vi "CalcAngle.vi"(10 "Octet 2":u8, 11 "Octet 1":u8) -> (3 "Angle":dbl)   [LabVIEW 2018]
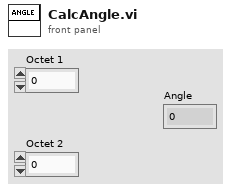
[diagram p1: front panel]
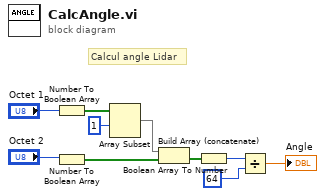
[diagram p0: block diagram]
diagram:
  # "Calcul angle Lidar"
  n1 = Number To Boolean Array(number="Octet 1") -> (Boolean array=w9:bool[])
  n2 = Number To Boolean Array(number="Octet 2") -> (Boolean array=w5:bool[])
  n3 = Array Subset(array=w9, index=1 ("indice")) -> (w6:bool[])  [unwired: 1 in]
  n4 = Build Array (concatenate)(w6, w5) -> (w4:bool[])
  n5 = Boolean Array To Number(Boolean array=w4) -> (number=w3:u32)
  n6 = Divide(x=w3, y=u32 64) -> (x/y=→"Angle":dbl)
